vi "FT_Read_String_Data.vi"(0 "Handle":u64, 1 "Bytes To Read":u32) -> (2 "FT_Status":u32(ring) items=["FT_OK", "FT_INVALID_HANDLE", "FT_DEVICE_NOT_FOUND", "FT_DEVICE_NOT_OPENED", "FT_IO_ERROR", "FT_INSUFFICIENT_RESOURCES", "FT_INVALID_PARAMETER", "FT_INVALID_BAUD_RATE", "FT_DEVICE_NOT_OPENED_FOR_ERASE", "FT_DEVICE_NOT_OPENED_FOR_WRITE", "FT_FAILED_TO_WRITE_DEVICE", "FT_EEPROM_READ_FAILED", "FT_EEPROM_WRITE_FAILED", "FT_EEPROM_ERASE_FAILED", "FT_EEPROM_NOT_PRESENT", "FT_EEPROM_NOT_PROGRAMMED", "FT_INVALID_ARGS", "FT_NOT_SUPPORTED", "FT_OTHER_ERROR"], 3 "Read Data":string, 4 "Bytes Read":u32)   [LabVIEW 2019, in "D2XX.lvlib"]
uses:
  D2XX.lvlib
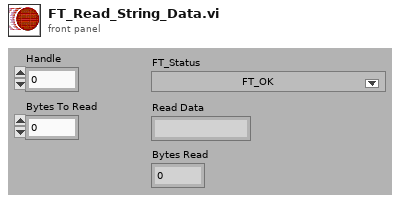
[diagram p1: front panel]
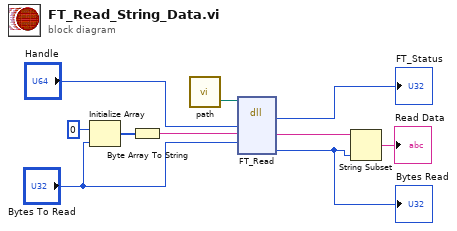
[diagram p0: block diagram]
diagram:
  n1 = Initialize Array(u8 0, "Bytes To Read") -> (w7:u8[])
  n2 = Byte Array To String(unsigned byte array=w7) -> (string=w6:string)
  n3 = call "path.vi"() -> ("lib path"=w1:path)
  n4 = dll-call lib="FTD2XX.dll" fn="FT_Read"(path in=w1, "Handle"="Handle", "Buffer"=w6, "BytesToRead"="Bytes To Read") -> (→"FT_Status":u32, "Buffer"=w3:string, "BytesReturned"=w2:u32)  [unwired: 5 in, 2 out]
  "Bytes Read" <- w2
  n5 = String Subset(string=w3, length (rest)=w2) -> (substring=→"Read Data":string)  [unwired: 1 in]
